vi "Start Sync.vi"(8 "error in (no error)":errorcluster, 11 "gRPC service in":refnum<class "OOBgRPCService.lvclass">) -> (0 "error out":errorcluster, 3 "gRPC service out":refnum<class "OOBgRPCService.lvclass">)   [LabVIEW 2025, in "OOB gRPC Server.lvlib" / "OOBgRPCService.lvclass"]
uses:
  OOBgRPCService.lvclass
  OOBgRPCService.lvclass/OOBgRPCService.ctl
  RPC Messages/hwval_GenericResponse.ctl
  RPC Messages/hwval_StatusResponse.ctl
  SubVIs/I2C Message Buffer - Dequeue.vi
  SubVIs/I2C Message Buffer - Check.vi
  OOB Data Transfer/OOB Data Transfer.lvlib
  OOB gRPC Server.lvlib
  I2C Bus Monitor.lvclass
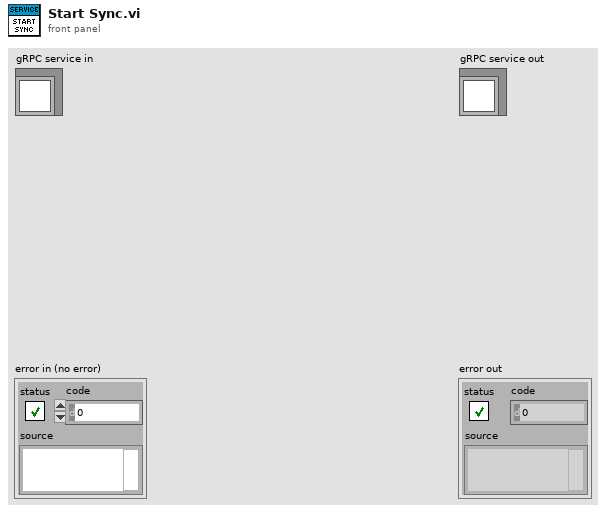
[diagram p1: front panel]
types:
  T1 = typedef "OOB gRPC Server.lvlib/hwval_GenericResponse.ctl" = cluster{"Payload":u8[]}
  T2 = typedef "OOB gRPC Server.lvlib/hwval_StatusResponse.ctl" = cluster{"Status":bool, "Code":i32, "Message":string}
  T3 = typedef "OOB gRPC Server.lvlib/OOBgRPCService.lvclass/Server Internal UEs.ctl" = cluster{"OOBgRPCService Generic Internal UE":refnum<user-event>, "OOBgRPCService PauseResume Internal UE":refnum<user-event>, "OOBgRPCService Export Internal UE":refnum<user-event>}
  T4 = typedef "OOB gRPC Server.lvlib/OOBgRPCService.lvclass/Server gRPC UEs.ctl" = cluster{"OOBgRPCService Generic gRPC UE":refnum<user-event>, "OOBgRPCService PauseResume gRPC UE":refnum<user-event>, "OOBgRPCService Export gRPC UE":refnum<user-event>}
  T5 = typedef "grpc-lvsupport-release.lvlib/grpcId.ctl" = u64
  T6 = typedef "OOB gRPC Server.lvlib/hwval_GenericRequest.ctl" = cluster{"Command":string, "Payload":u8[]}
  T7 = typedef "OOB Data Transfer.lvlib/OOB to Logic Data.ctl" = cluster{"PauseResume":bool, "Export":string, "Scan Bus":bool, "I2C Script":cluster{"Send":bool, "Path":string}, "I2C CMD":cluster{"Send":bool, "SLAVE ADDR.":u8, "REG. ADDR.":u16, "DATA":u8, "R/W":bool}}
  T8 = cluster{"Send":bool, "SLAVE ADDR.":u8, "REG. ADDR.":u16, "DATA":u8, "R/W":bool}
  T9 = typedef "OOB gRPC Server.lvlib/hwval_BoolRequest.ctl" = cluster{"BooleanData":bool}
  T10 = typedef "OOB gRPC Server.lvlib/hwval_ExportRequest.ctl" = cluster{"FileType":string}
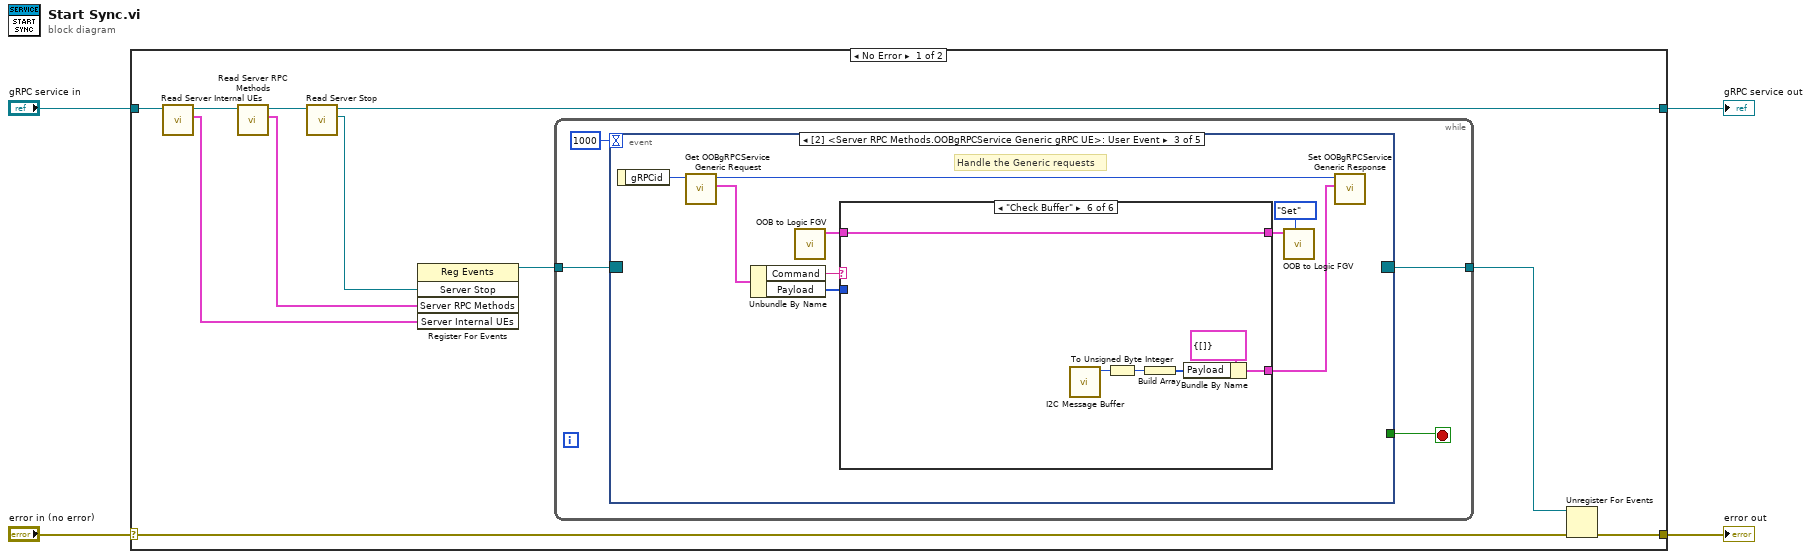
[diagram p0: block diagram]
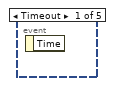
[diagram p2: hidden frame]
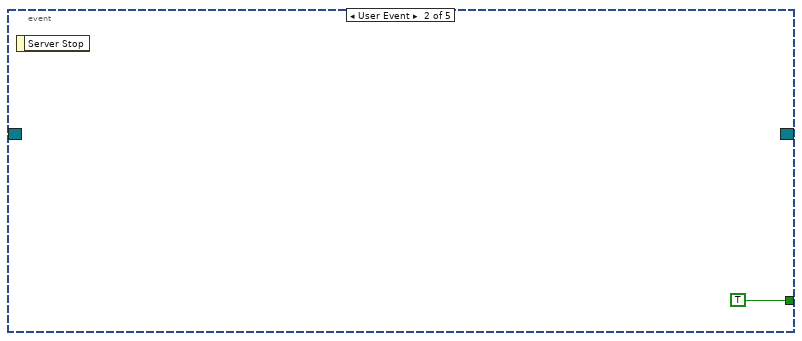
[diagram p3: hidden frame]
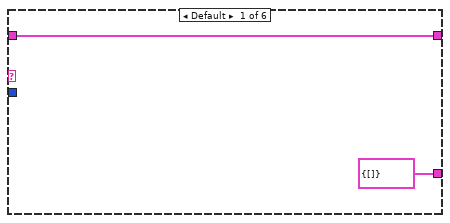
[diagram p4: hidden frame]
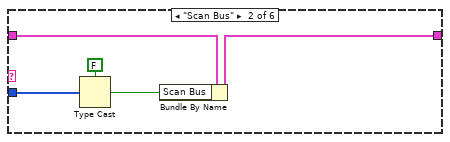
[diagram p5: hidden frame]
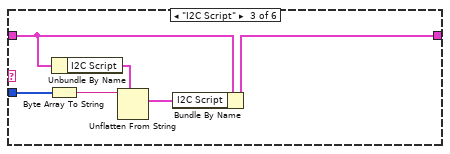
[diagram p6: hidden frame]
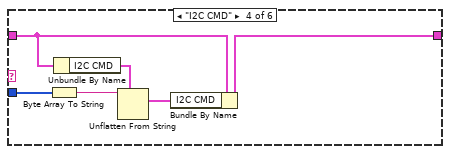
[diagram p7: hidden frame]
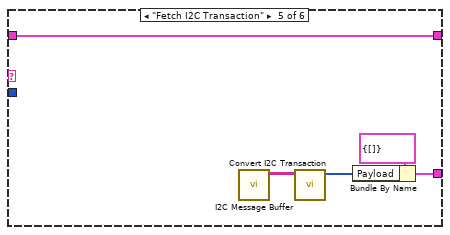
[diagram p8: hidden frame]
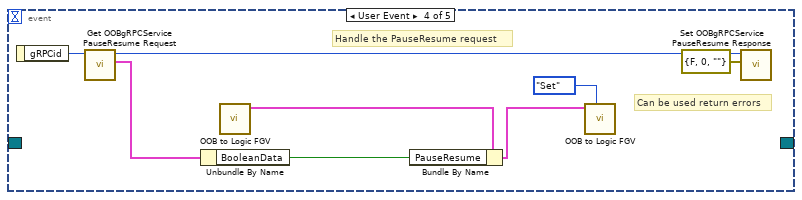
[diagram p9: hidden frame]
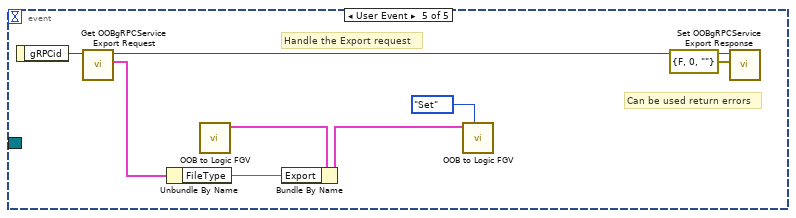
[diagram p10: hidden frame]
diagram:
  n1 = case shown="No Error" "error in (no error)" {
    selector: "error in (no error)" -> [w9 w77]
    tunnel: [w8 w77] -> w3
    tunnel: [w6 w76] -> w1
    tunnel: "gRPC service in" -> [w15 w76]
    frame No Error {
      n2 = call "Read Server Internal UEs.vi"("gRPC service in"=w15) -> ("Server Internal UEs"=w13:T3, "gRPC service out"=w14:refnum<class "OOBgRPCService.lvclass">)  [unwired: 8 in, 1 out]
      n3 = call "Read Server RPC Methods.vi"("gRPC service in"=w14) -> ("Server RPC Methods"=w7:T4, "gRPC service out"=w12:refnum<class "OOBgRPCService.lvclass">)  [unwired: 8 in, 1 out]
      n4 = call-dynamic "Read Server Stop.vi"("gRPC service in"=w12) -> ("Server Stop"=w5:refnum<user-event>, "gRPC service out"=w6:refnum<class "OOBgRPCService.lvclass">)  [unwired: 8 in, 1 out]
      n5 = register-events(w5, w7, w13) -> (reference out=w11:refnum<event-registration>)  [unwired: 2 in, 1 out]
      n6 = while {
        tunnel: w11 -> [w19]
        tunnel: [w17] -> w10
        stop <- w18 stop-if-true
        n7 = event "RPC Methods Event Structure" shown="[2] <Server RPC Methods.OOBgRPCService Generic gRPC UE>: User Event" {
          selector: w19 -> [_ _ _ _ _]
          dyn-events: [_ _ _ _ _] -> w17
          timeout: 1000 -> [_ _ _ _ _]
          tunnel: [_ TRUE _ _ _] -> w18
          event Timeout {
            n8 = event-data() -> ()  [unwired: 1 in, 1 out]
          }
          event User Event {
            n9 = event-data() -> ()  [unwired: 1 in, 1 out]
          }
          event User Event {
            # "Handle the Generic requests"
            n10 = event-data() -> ("gRPCid"=w29:T5)  [unwired: 1 in]
            n11 = call "Get OOBgRPCService Generic Request.vi"("gRPCid"=w29) -> ("Message Data"=w28:T6, "gRPCid out"=w21:T5)  [unwired: 8 in, 1 out]
            n12 = Unbundle By Name(w28) -> ("Command"=w24:string, "Payload"=w23:u8[])
            n13 = call "OOB to Logic FGV.vi"() -> ("OOB to Logic Data out"=w26:T7)  [unwired: 10 in, 1 out]
            n14 = case shown="\"Check Buffer\"" w24 {
              tunnel: w26 -> [w31 w36 w39 w45 w53 w59]
              tunnel: [w31 w35 w42 w48 w53 w59] -> w25
              tunnel: w23 -> [_ w34 w41 w47 _ _]
              tunnel: [T1 {"Payload"=[]} ("Message Data") _ _ _ w51 w57] -> w22
              frame Default {
              }
              frame "Scan Bus" {
                n15 = Type Cast(type=FALSE, x=w34) -> (*(type *) &x=w33:bool)
                n16 = Bundle By Name(cluster=w36, "Scan Bus"=w33) -> (w35:T7)
              }
              frame "I2C Script" {
                n17 = Byte Array To String(unsigned byte array=w41) -> (string=w40:string)
                n18 = Unbundle By Name(w39) -> ("I2C Script"=w38:cluster{"Send":bool, "Path":string})
                n19 = Unflatten From String(type=w38, binary string=w40) -> (value=w37:cluster{"Send":bool, "Path":string})  [unwired: 3 in, 2 out]
                n20 = Bundle By Name(cluster=w39, "I2C Script"=w37) -> (w42:T7)
              }
              frame "I2C CMD" {
                n21 = Byte Array To String(unsigned byte array=w47) -> (string=w46:string)
                n22 = Unbundle By Name(w45) -> ("I2C CMD"=w44:T8)
                n23 = Unflatten From String(type=w44, binary string=w46) -> (value=w43:T8)  [unwired: 3 in, 2 out]
                n24 = Bundle By Name(cluster=w45, "I2C CMD"=w43) -> (w48:T7)
              }
              frame "Fetch I2C Transaction" {
                n25 = call-poly "I2C Message Buffer.vi"() -> ("I2C Transaction"=w49:string[][])  [unwired: 10 in, 1 out]
                n26 = call "Convert I2C Transaction.vi"("I2C Transaction"=w49) -> ("U8 Array"=w50:u8[])  [unwired: 9 in, 1 out]
                n27 = Bundle By Name(cluster=T1 {"Payload"=[]} ("Message Data"), "Payload"=w50) -> (w51:T1)
              }
              frame "Check Buffer" {
                n28 = call-poly "I2C Message Buffer.vi"() -> ("Transactions"=w56:i32)  [unwired: 9 in, 2 out]
                n29 = To Unsigned Byte Integer(number=w56) -> (unsigned 8bit integer=w54:u8)
                n30 = Build Array(w54) -> (w55:u8[])
                n31 = Bundle By Name(cluster=T1 {"Payload"=[]} ("Message Data"), "Payload"=w55) -> (w57:T1)
              }
            }
            n32 = call "OOB to Logic FGV.vi"("Op (Get)"=enum16{"Get", "Set"}."Set", "OOB to Logic Data in"=w25) -> ()  [unwired: 8 in, 2 out]
            n33 = call "Set OOBgRPCService Generic Response.vi"("Message Data"=w22, "gRPCid in"=w21) -> ()  [unwired: 9 in, 1 out]
          }
          event User Event {
            # "Handle the PauseResume request"
            # "Can be used return errors"
            n34 = event-data() -> ("gRPCid"=w61:T5)  [unwired: 1 in]
            n35 = call "Get OOBgRPCService PauseResume Request.vi"("gRPCid"=w61) -> ("Message Data"=w63:T9, "gRPCid out"=w64:T5)  [unwired: 8 in, 1 out]
            n36 = Unbundle By Name(w63) -> ("BooleanData"=w62:bool)
            n37 = call "OOB to Logic FGV.vi"() -> ("OOB to Logic Data out"=w66:T7)  [unwired: 10 in, 1 out]
            n38 = Bundle By Name(cluster=w66, "PauseResume"=w62) -> (w65:T7)
            n39 = call "OOB to Logic FGV.vi"("Op (Get)"=enum16{"Get", "Set"}."Set", "OOB to Logic Data in"=w65) -> ()  [unwired: 8 in, 2 out]
            n40 = call "Set OOBgRPCService PauseResume Response.vi"("Message Data"=T2 {"Status"=FALSE, "Code"=0, "Message"=""}, "gRPCid in"=w64) -> ()  [unwired: 9 in, 1 out]
          }
          event User Event {
            # "Handle the Export request"
            # "Can be used return errors"
            n41 = event-data() -> ("gRPCid"=w69:T5)  [unwired: 1 in]
            n42 = call "Get OOBgRPCService Export Request.vi"("gRPCid"=w69) -> ("Message Data"=w71:T10, "gRPCid out"=w75:T5)  [unwired: 8 in, 1 out]
            n43 = Unbundle By Name(w71) -> ("FileType"=w70:string)
            n44 = call "OOB to Logic FGV.vi"() -> ("OOB to Logic Data out"=w73:T7)  [unwired: 10 in, 1 out]
            n45 = Bundle By Name(cluster=w73, "Export"=w70) -> (w72:T7)
            n46 = call "OOB to Logic FGV.vi"("Op (Get)"=enum16{"Get", "Set"}."Set", "OOB to Logic Data in"=w72) -> ()  [unwired: 8 in, 2 out]
            n47 = call "Set OOBgRPCService Export Response.vi"("Message Data"=T2 {"Status"=FALSE, "Code"=0, "Message"=""}, "gRPCid in"=w75) -> ()  [unwired: 9 in, 1 out]
          }
        }
      }
      n48 = Unregister For Events(event registration refnum=w10, error in=w9) -> (error out=w8:errorcluster)
    }
    frame Error {
    }
  }
  "error out" <- w3
  "gRPC service out" <- w1
